vi "RemoteVI VI Stopped.vi"(0 "VI":refnum<vi>, 1 "window":u64, 5 "last check":u32, 7 "VI Server ok?":bool=TRUE) -> (4 "stopped?":bool, 6 "last check out":u32)   [LabVIEW 2020, in "RemoteVI.lvlib"]
doc: "Checks once a second whether the published VI has stopped: when VI Server may be called (VI Server ok? - no popup open, no recent click) and 1000 ms have passed since last check, asks RemoteVI Target Running.vi; stopped? is TRUE when VI is idle or bad or its state cannot be read, or - for a window target - when the window no longer exists. Otherwise stopped? is FALSE and nothing is read. So the server ends with your application."
uses:
  RemoteVI.lvlib
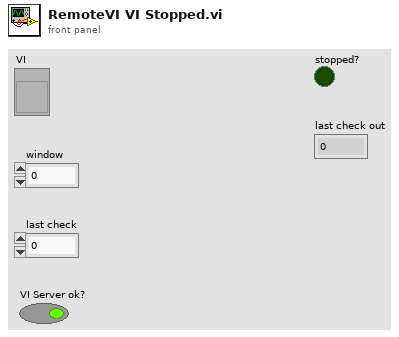
[diagram p1: front panel]
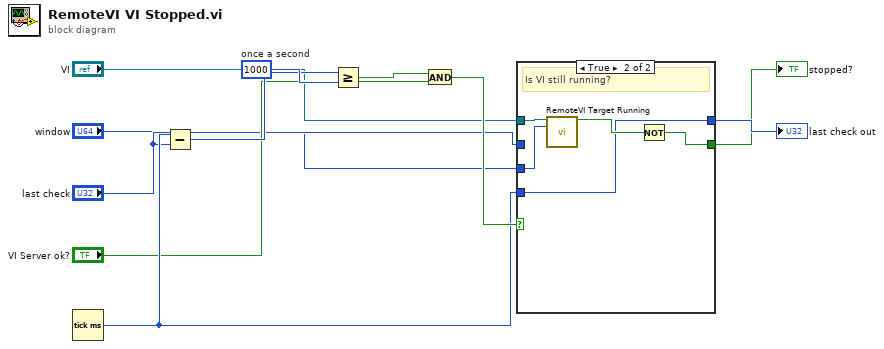
[diagram p0: block diagram]
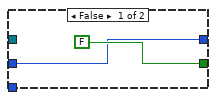
[diagram p2: hidden frame]
diagram:
  w7 = u32 1000  # once a second
  n1 = Tick Count (ms)() -> (millisecond timer value=w5:u32)
  n2 = Subtract(x=w5, y="last check") -> (x-y=w6:u32)
  n3 = Greater Or Equal?(x=w6, y=w7) -> (x >= y?=w8:bool)
  n4 = And(x=w8, y="VI Server ok?") -> (x .and. y?=w9:bool)
  n5 = case shown="True" w9 {
    tunnel: "VI" -> [_ w14]
    tunnel: "last check" -> [w12 _]
    tunnel: "window" -> [_ w16]
    tunnel: w5 -> [_ w15]
    tunnel: [w12 w15] -> w11
    tunnel: [FALSE w18] -> w10
    frame False {
    }
    frame True {
      # "Is VI still running?"
      n6 = call "RemoteVI Target Running.vi"("VI"=w14, "window"=w16) -> ("running?"=w17:bool)  [unwired: 13 in]
      n7 = Not(x=w17) -> (.not. x?=w18:bool)
    }
  }
  "stopped?" <- w10
  "last check out" <- w11
